vi "Display.vi"(0 "Data":dbl[](array[numeric]), 2 "dt":dbl, 3 "t0":timestamp, 6 "索引 1":i32, 7 "索引 3":i32, 8 "索引 2":i32, 9 "索引 4":i32) -> (10 "输出波形 1":waveform(dbl), 11 "输出波形 3":waveform(dbl), 12 "输出波形 2":waveform(dbl), 13 "输出波形 4":waveform(dbl), 14 "输出波形 5":waveform(dbl), 15 "输出波形 6":waveform(dbl), 16 "输出波形 7":waveform(dbl), 17 "输出波形 8":waveform(dbl), 18 "输出波形 Ch1":waveform(dbl), 19 "输出波形 Ch2":waveform(dbl))   [LabVIEW 2026, in "UI-温度采集.lvlib"]
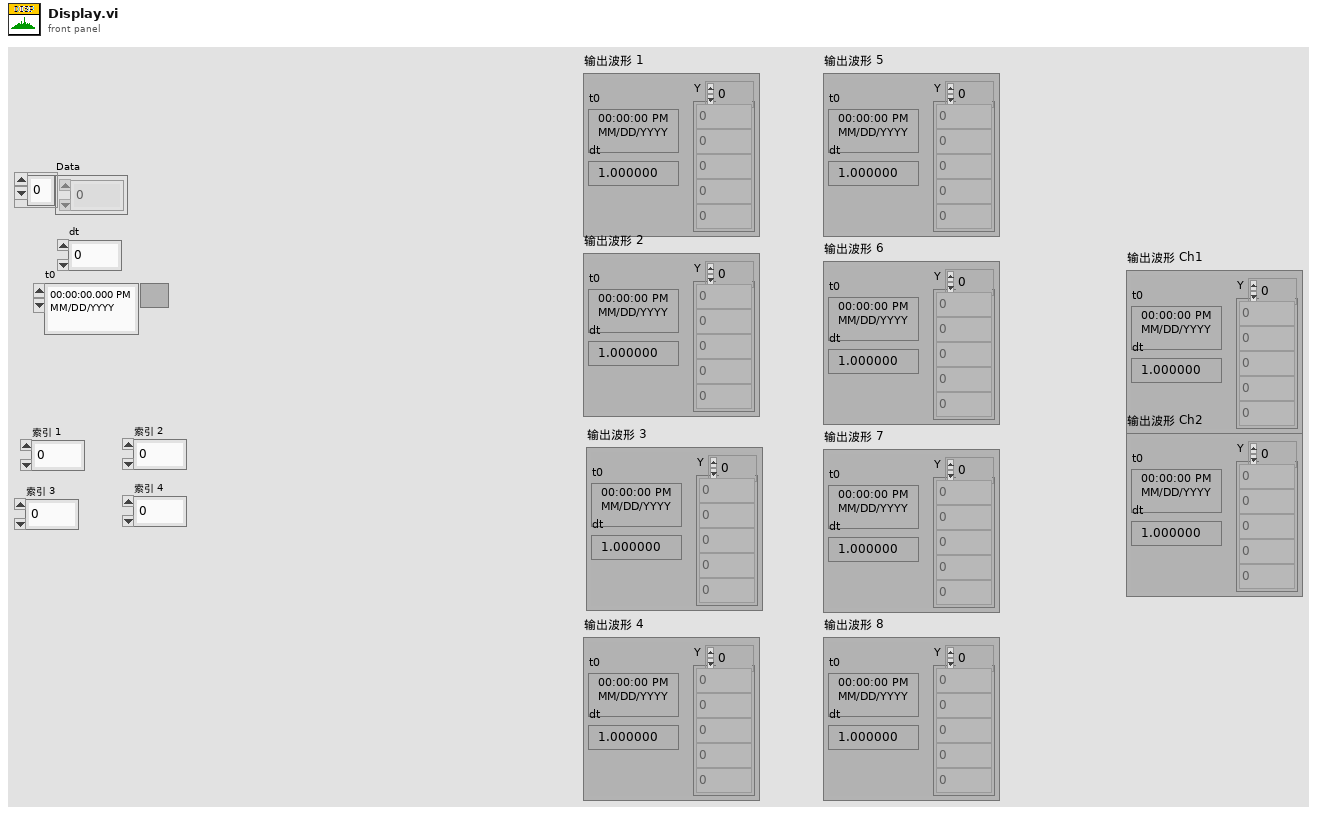
[diagram p1: front panel]
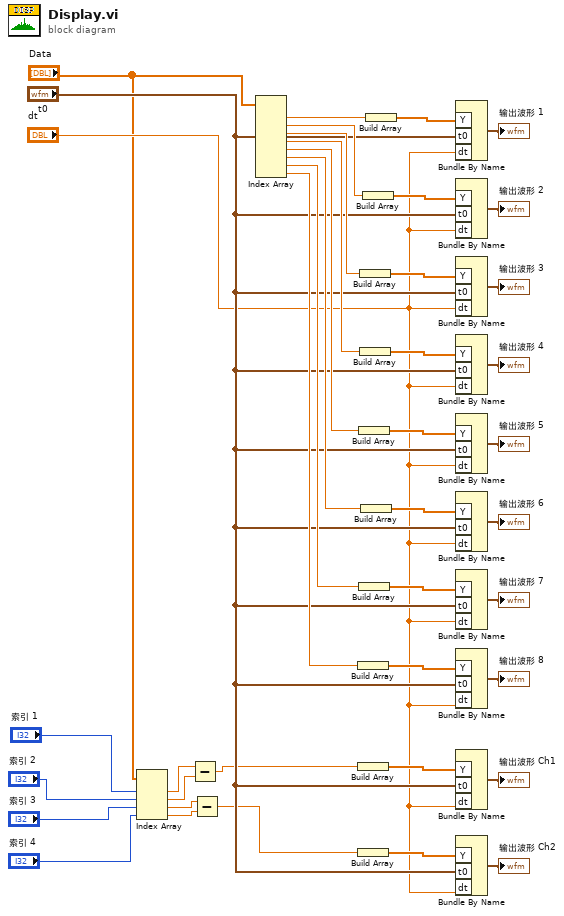
[diagram p0: block diagram]
diagram:
  n1 = Index Array(array="Data", index #1="索引 1", index #2="索引 2", index #3="索引 3", index #4="索引 4") -> (element #1=w21:dbl, element #2=w20:dbl, element #3=w19:dbl, element #4=w18:dbl)
  n2 = Subtract(x=w21, y=w20) -> (x-y=w15:dbl)
  n3 = Subtract(x=w19, y=w18) -> (x-y=w16:dbl)
  n4 = Index Array(array="Data") -> (element #1=w41:dbl, element #2=w38:dbl, element #3=w36:dbl, element #4=w34:dbl, element #5=w29:dbl, element #6=w28:dbl, element #7=w27:dbl, element #8=w24:dbl)  [unwired: 8 in]
  n5 = Build Array(w24) -> (w30:dbl[])
  n6 = Build Array(w15) -> (w26:dbl[])
  n7 = Build Array(w16) -> (w25:dbl[])
  n8 = Build Array(w29) -> (w33:dbl[])
  n9 = Build Array(w27) -> (w31:dbl[])
  n10 = Build Array(w36) -> (w37:dbl[])
  n11 = Build Array(w34) -> (w35:dbl[])
  n12 = Build Array(w28) -> (w32:dbl[])
  n13 = Build Array(w38) -> (w39:dbl[])
  n14 = Build Array(w41) -> (w40:dbl[])
  n15 = Bundle By Name("Y"=w40, "t0"="t0", "dt"="dt") -> (→"输出波形 1":waveform(dbl))  [unwired: 1 in]
  n16 = Bundle By Name("Y"=w39, "t0"="t0", "dt"="dt") -> (→"输出波形 2":waveform(dbl))  [unwired: 1 in]
  n17 = Bundle By Name("Y"=w37, "t0"="t0", "dt"="dt") -> (→"输出波形 3":waveform(dbl))  [unwired: 1 in]
  n18 = Bundle By Name("Y"=w35, "t0"="t0", "dt"="dt") -> (→"输出波形 4":waveform(dbl))  [unwired: 1 in]
  n19 = Bundle By Name("Y"=w33, "t0"="t0", "dt"="dt") -> (→"输出波形 5":waveform(dbl))  [unwired: 1 in]
  n20 = Bundle By Name("Y"=w32, "t0"="t0", "dt"="dt") -> (→"输出波形 6":waveform(dbl))  [unwired: 1 in]
  n21 = Bundle By Name("Y"=w31, "t0"="t0", "dt"="dt") -> (→"输出波形 7":waveform(dbl))  [unwired: 1 in]
  n22 = Bundle By Name("Y"=w30, "t0"="t0", "dt"="dt") -> (→"输出波形 8":waveform(dbl))  [unwired: 1 in]
  n23 = Bundle By Name("Y"=w26, "t0"="t0", "dt"="dt") -> (→"输出波形 Ch1":waveform(dbl))  [unwired: 1 in]
  n24 = Bundle By Name("Y"=w25, "t0"="t0", "dt"="dt") -> (→"输出波形 Ch2":waveform(dbl))  [unwired: 1 in]
